vi "List Available Measurements.vi"(8 "error in (no error)":errorcluster, 10 "enumerate services request":T1, 11 "multicolumnListbox ref in":refnum<vi>) -> (0 "error out":errorcluster, 1 "warning":string, 2 "available measurement details":T2, 3 "multicolumnListbox ref":refnum<vi>)   [LabVIEW 2021, in "MeasurementClient Editor.lvlib"]
uses:
  MeasurementClient Editor.lvlib
  <vilib>/gRPC/Generated APIs/ni/measurementlink/discovery/v1/RPC Messages/ni_measurementlink_discovery_v1_EnumerateServicesResponse.ctl
  <vilib>/gRPC/Generated APIs/ni/measurementlink/discovery/v1/RPC Messages/ni_measurementlink_discovery_v1_ServiceDescriptor.ctl
  <vilib>/gRPC/Generated APIs/ni/measurementlink/discovery/v1/RPC Messages/ni_measurementlink_discovery_v1_ServiceDescriptor_AnnotationsEntry.ctl
  <vilib>/gRPC/Generated APIs/ni/measurementlink/discovery/v1/RPC Messages/ni_measurementlink_discovery_v1_EnumerateServicesRequest.ctl
  <vilib>/Utility/miscctls.llb/LVRowAndColumnTypeDef.ctl
  <vilib>/Plug-In SDKs/Clients/Discovery V1/NI Discovery V1 Client.lvlib
  <vilib>/gRPC/Generated APIs/ni/measurementlink/discovery/v1/ni.measurementlink.discovery.v1.api.lvlib
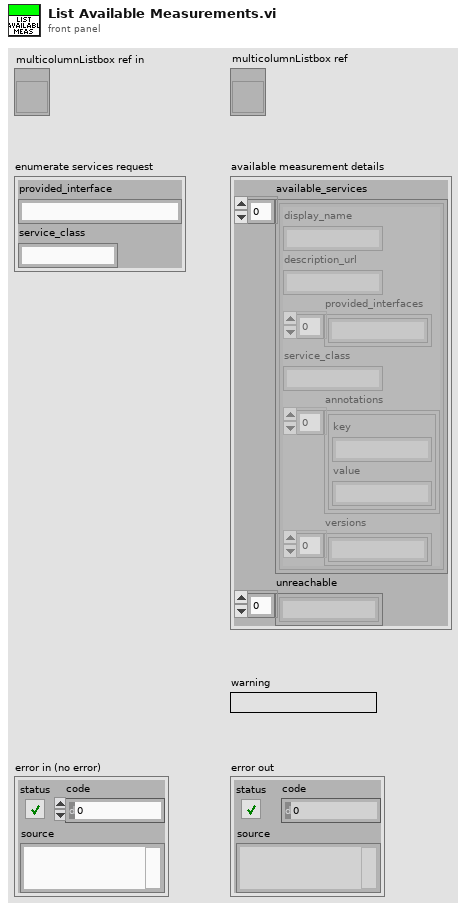
[diagram p1: front panel]
types:
  T1 = typedef "ni.measurementlink.discovery.v1.api.lvlib/ni_measurementlink_discovery_v1_EnumerateServicesRequest.ctl" = cluster{"provided_interface":string, "service_class":string}
  T2 = typedef "ni.measurementlink.discovery.v1.api.lvlib/ni_measurementlink_discovery_v1_EnumerateServicesResponse.ctl" = cluster{"available_services":T3[], "unreachable":string[]}
  T3 = typedef "ni.measurementlink.discovery.v1.api.lvlib/ni_measurementlink_discovery_v1_ServiceDescriptor.ctl" = cluster{"display_name":string, "description_url":string, "provided_interfaces":string[], "service_class":string, "annotations":T4[], "versions":string[]}
  T4 = typedef "ni.measurementlink.discovery.v1.api.lvlib/ni_measurementlink_discovery_v1_ServiceDescriptor_AnnotationsEntry.ctl" = cluster{"key":string, "value":string}
  T5 = typedef "LVRowAndColumnTypeDef.ctl" = cluster{"Row":i32, "Column":i32}
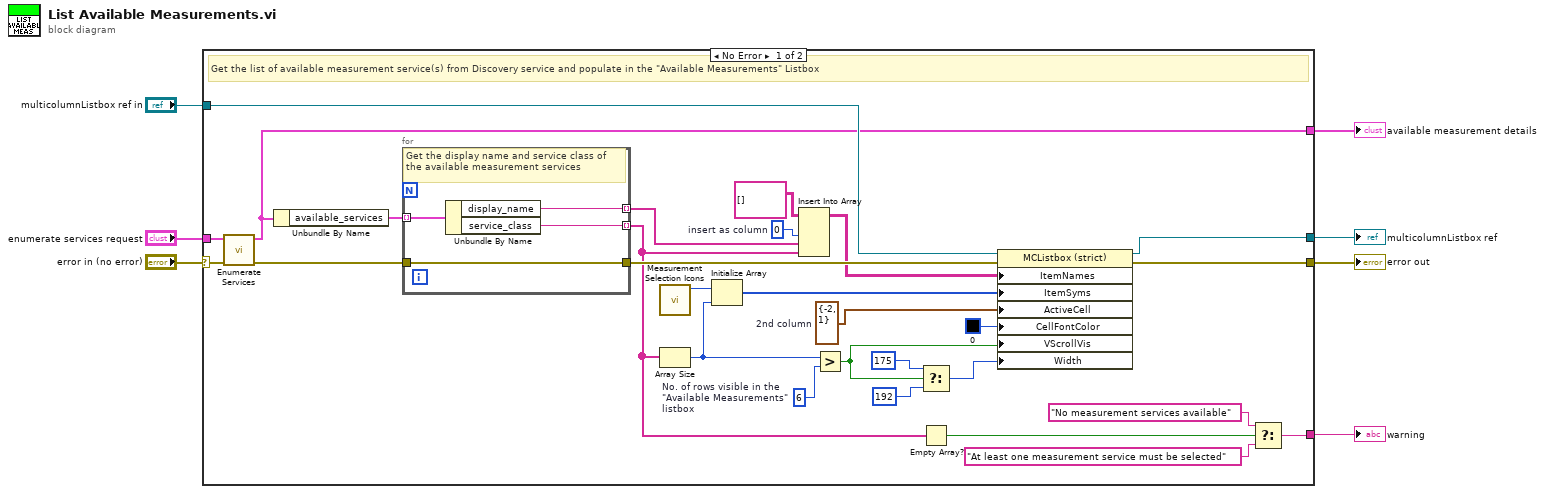
[diagram p0: block diagram]
diagram:
  n1 = case shown="No Error" "error in (no error)" {
    selector: "error in (no error)" -> [w30 w40]
    tunnel: [w12 w40] -> w7
    tunnel: "multicolumnListbox ref in" -> [w34 w41]
    tunnel: [w13 w41] -> w5
    tunnel: [w33 _] -> w4
    tunnel: [w29 _] -> w2
    tunnel: "enumerate services request" -> [w28 _]
    frame No Error {
      w15 = T5 {"Row"=-2, "Column"=1}  # 2nd column
      w22 = 0  # insert as column
      w31 = 6  # No. of rows visible in the "Available Measurements" listbox
      # "Get the list of available measurement service(s) from Discovery service and populate in the \"Available Measurements\" Listbox"
      n2 = call <vilib>:"Enumerate Services.vi"("error in"=w30, "request data"=w28) -> ("error out"=w26:errorcluster, "response data"=w29:T2)  [unwired: 7 in]
      n3 = Unbundle By Name(w29) -> ("available_services"=w23:T3[])
      n4 = for {
        tunnel: w23 -> [w39] mode=indexing
        tunnel: [w38] -> w16 mode=indexing
        tunnel: [w36] -> w35
        tunnel: w26 -> [w36]
        tunnel: [w37] -> w18 mode=indexing
        # "Get the display name and service class of the available measurement services"
        n5 = Unbundle By Name(w39) -> ("display_name"=w37:string, "service_class"=w38:string)
      }
      n6 = call "Measurement Selection Icons.vi"() -> ("Unchecked"=w21:i32)  [unwired: 10 in, 1 out]
      n7 = Array Size(array=w16) -> (size(s)=w20:i32)
      n8 = Initialize Array(w21, w20) -> (w19:i32[])
      n9 = Insert Into Array(array=string[][] [], index (col)=w22, new element #1=w18, new element #2=w16) -> (w24:string[][])  [unwired: 1 in]
      n10 = Greater?(x=w20, y=w31) -> (0:w11:bool)
      n11 = Select(t=u32 175 ("Active Cell:Cell Size:Width"), s=w11, f=u32 192 ("Active Cell:Cell Size:Width")) -> (s? t:f=w8:u32)
      n12 = Empty Array?(array=w16) -> (empty?=w17:bool)
      n13 = property class="MCListbox (strict)"(reference=w34, error in=w35, "ItemNames"=w24, "ItemSyms"=w19, "ActiveCell"=w15, "CellFontColor"=u32 0 ("Active Cell:Cell Font:Color"), "VScrollVis"=w11, "Width"=w8) -> (reference out=w13:refnum<vi>, error out=w12:errorcluster)
      n14 = Select(t="No measurement services available", s=w17, f="At least one measurement service must be selected") -> (s? t:f=w33:string)
    }
    frame Error {
      # "Pass"
    }
  }
  "error out" <- w7
  "multicolumnListbox ref" <- w5
  "warning" <- w4
  "available measurement details" <- w2
